vi "Parse LabVIEWCLI Argument.vi"(6 "Default":string, 8 "error in":errorcluster, 9 "Optional":bool, 10 "Identifier":string, 11 "Args":string[](array[string])) -> (0 "error out":errorcluster, 2 "Value":string, 3 "Found":bool)   [LabVIEW 2026]
doc: "This VI parses the provided parameter from the argument array. The identifier must include the parameter prefix. If a parameter is not found and the boolean input <i>Optional</i> is false, the VI will produce an error."
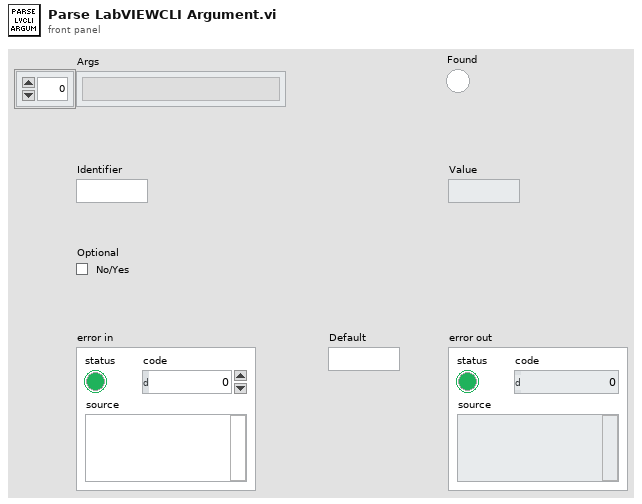
[diagram p1: front panel]
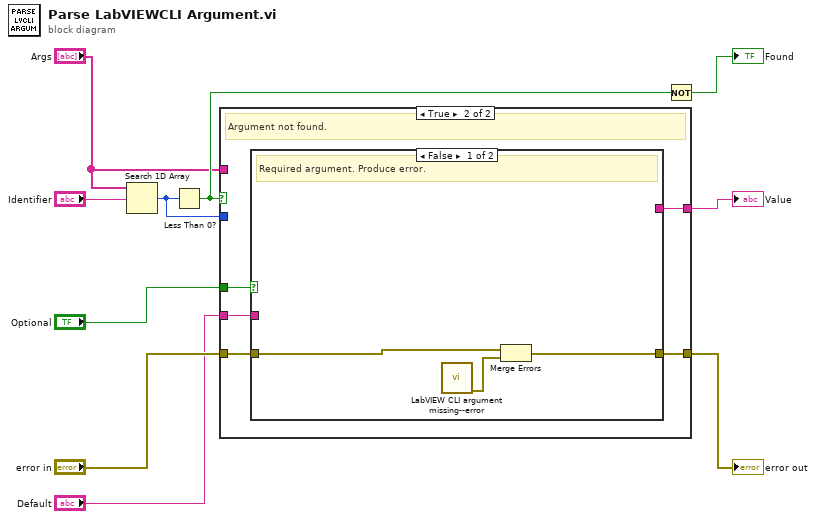
[diagram p0: block diagram]
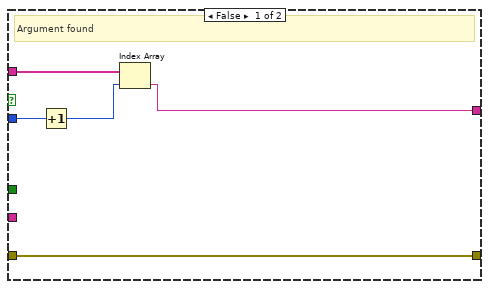
[diagram p2: hidden frame]
diagram:
  n1 = Search 1D Array(1D array="Args", element="Identifier") -> (index of element=w4:i32)  [unwired: 1 in]
  n2 = Less Than 0?(x=w4) -> (x < 0?=w5:bool)
  n3 = case shown="True" w5 {
    tunnel: "Optional" -> [_ w18]
    tunnel: "error in" -> [w15 w20]
    tunnel: [w15 w19] -> w9
    tunnel: w4 -> [w14 _]
    tunnel: "Args" -> [w13 _]
    tunnel: [w11 w17] -> w2
    tunnel: "Default" -> [_ w16]
    frame False {
      # "Argument found"
      n4 = Increment(x=w14) -> (x+1=w12:i32)
      n5 = Index Array(array=w13, index=w12) -> (element=w11:string)
    }
    frame True {
      # "Argument not found."
      n6 = case shown="False" w18 {
        tunnel: w20 -> [w23 w25]
        tunnel: [w21 w25] -> w19
        tunnel: [_ w24] -> w17
        tunnel: w16 -> [_ w24]
        frame False {
          # "Required argument. Produce error."
          n7 = call "LabVIEW CLI argument missing--error.vi"() -> ("error out"=w22:errorcluster)  [unwired: 11 in]
          n8 = Merge Errors(w23, w22) -> (w21:errorcluster)
        }
        frame True {
          # "Argument is optional."
        }
      }
    }
  }
  "Value" <- w2
  "error out" <- w9
  n9 = Not(x=w5) -> (.not. x?=→"Found":bool)
